vi "Game_Board_Click.vi"(0 "Context":T1={"Screen"=enum."Settings", "Settings"=[0, 0, 1, 1], "Board"={"Grid"=array15x15[225 elements], "Move History"=[], "Last Move"={"Row"=-1, "Col"=-1, "Stone"=enum."Empty"}}, "Status"=enum."Idle", "Game ID"=0, "Player Stone"=enum."Black", "Hover"={"Row"=-1, "Col"=-1, "Stone"=enum."Empty"}, "Hover Button"=-1, "Win Line"=[], "Score 1"=0, "Score 2"=0, "Draws"=0, "Status Text"="", "Status Color"=0}, 5 "Row":i32=-1, 7 "Col":i32=-1, 11 "error in":errorcluster) -> (4 "Context out":T1={"Screen"=enum."Settings", "Settings"=[0, 0, 1, 1], "Board"={"Grid"=array15x15[225 elements], "Move History"=[], "Last Move"={"Row"=-1, "Col"=-1, "Stone"=enum."Empty"}}, "Status"=enum."Idle", "Game ID"=0, "Player Stone"=enum."Black", "Hover"={"Row"=-1, "Col"=-1, "Stone"=enum."Empty"}, "Hover Button"=-1, "Win Line"=[], "Score 1"=0, "Score 2"=0, "Draws"=0, "Status Text"="", "Status Color"=0}, 6 "Need AI":bool, 15 "error out":errorcluster)   [LabVIEW 2026]
doc: "바둑판 (Row,Col) 클릭 처리. 2인 플레이는 수순(짝/홀)으로 흑/백 결정, AI 대전은 Player Stone.\n승/무/금수/차례 문구와 점수를 갱신하고, AI 대전에서 게임이 계속되면 Need AI = True."
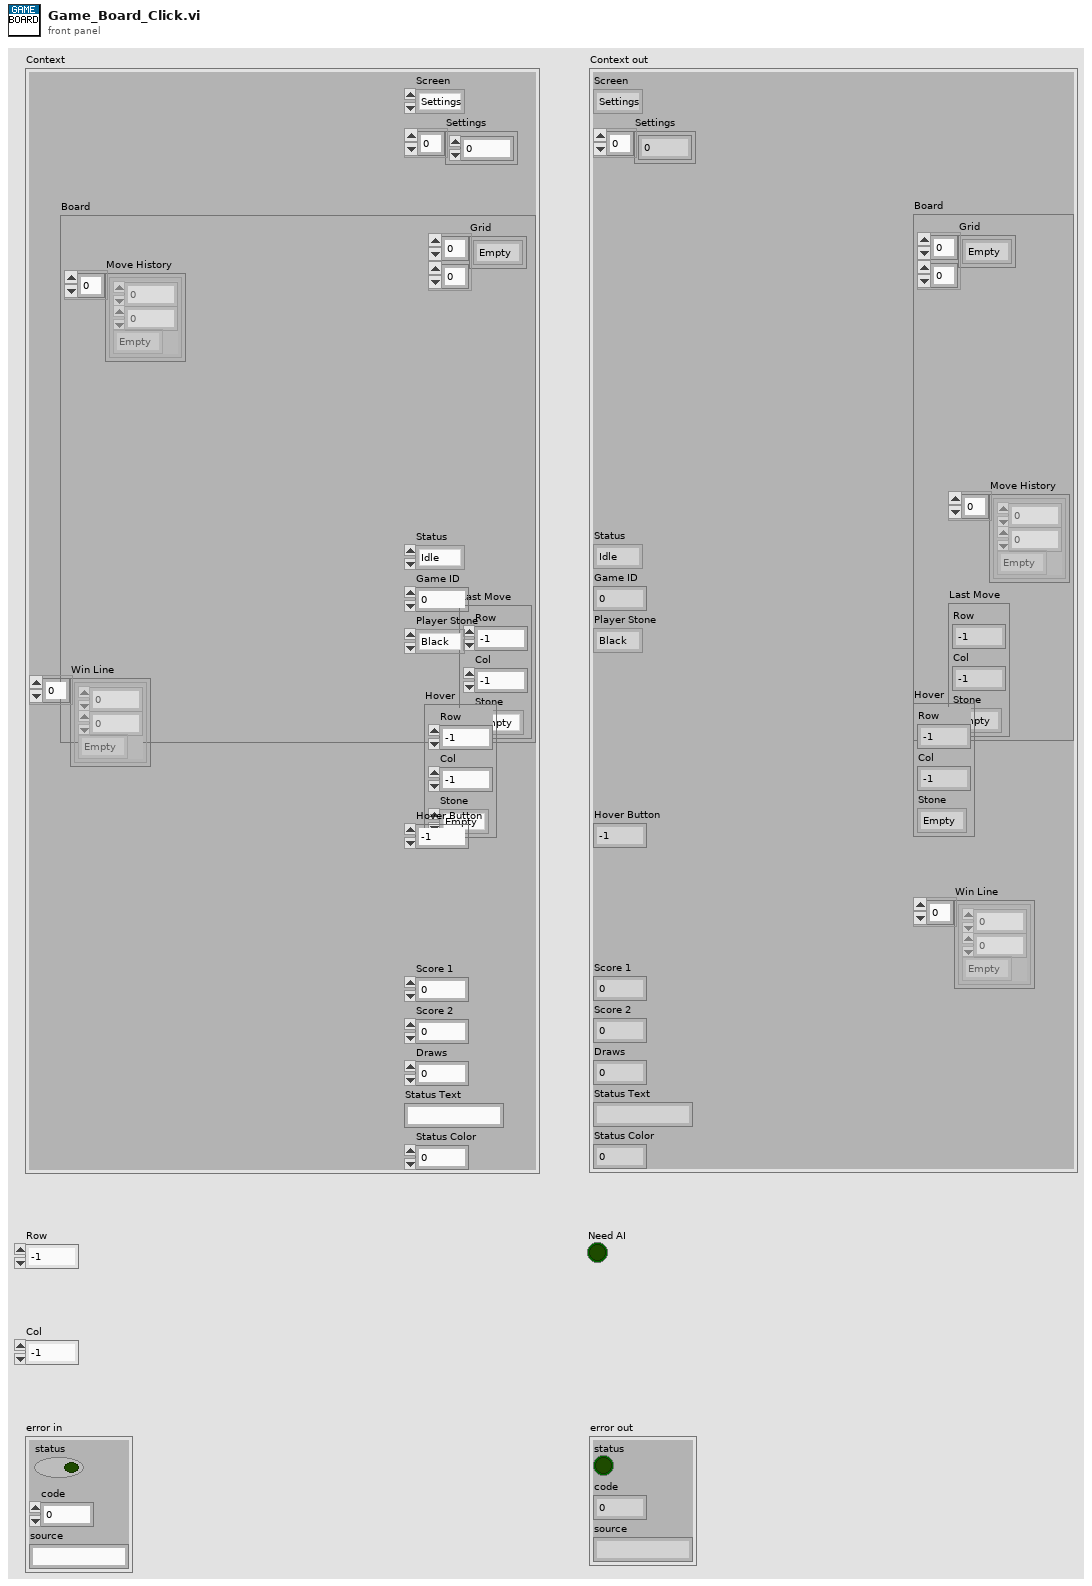
[diagram p1: front panel]
types:
  T1 = cluster{"Screen":enum16{"Settings", "Game"}, "Settings":i32[], "Board":cluster{"Grid":enum8{"Empty", "Black", "White"}[][], "Move History":cluster{"Row":i32, "Col":i32, "Stone":enum8{"Empty", "Black", "White"}}[], "Last Move":cluster{"Row":i32, "Col":i32, "Stone":enum8{"Empty", "Black", "White"}}}, "Status":enum16{"Idle", "Player Turn", "AI Thinking", "Game Over"}, "Game ID":u32, "Player Stone":enum8{"Empty", "Black", "White"}, "Hover":cluster{"Row":i32, "Col":i32, "Stone":enum8{"Empty", "Black", "White"}}, "Hover Button":i32, "Win Line":cluster{"Row":i32, "Col":i32, "Stone":enum8{"Empty", "Black", "White"}}[], "Score 1":i32, "Score 2":i32, "Draws":i32, "Status Text":string, "Status Color":u32}
  T2 = enum16{"Idle", "Player Turn", "AI Thinking", "Game Over"}
  T3 = cluster{"Row":i32, "Col":i32, "Stone":enum8{"Empty", "Black", "White"}}
  T4 = enum8{"None", "Double Three", "Double Four", "Overline"}
  T5 = cluster{"Grid":enum8{"Empty", "Black", "White"}[][], "Move History":cluster{"Row":i32, "Col":i32, "Stone":enum8{"Empty", "Black", "White"}}[], "Last Move":cluster{"Row":i32, "Col":i32, "Stone":enum8{"Empty", "Black", "White"}}}
  T6 = cluster{"Row":i32, "Col":i32, "Stone":enum8{"Empty", "Black", "White"}}[]
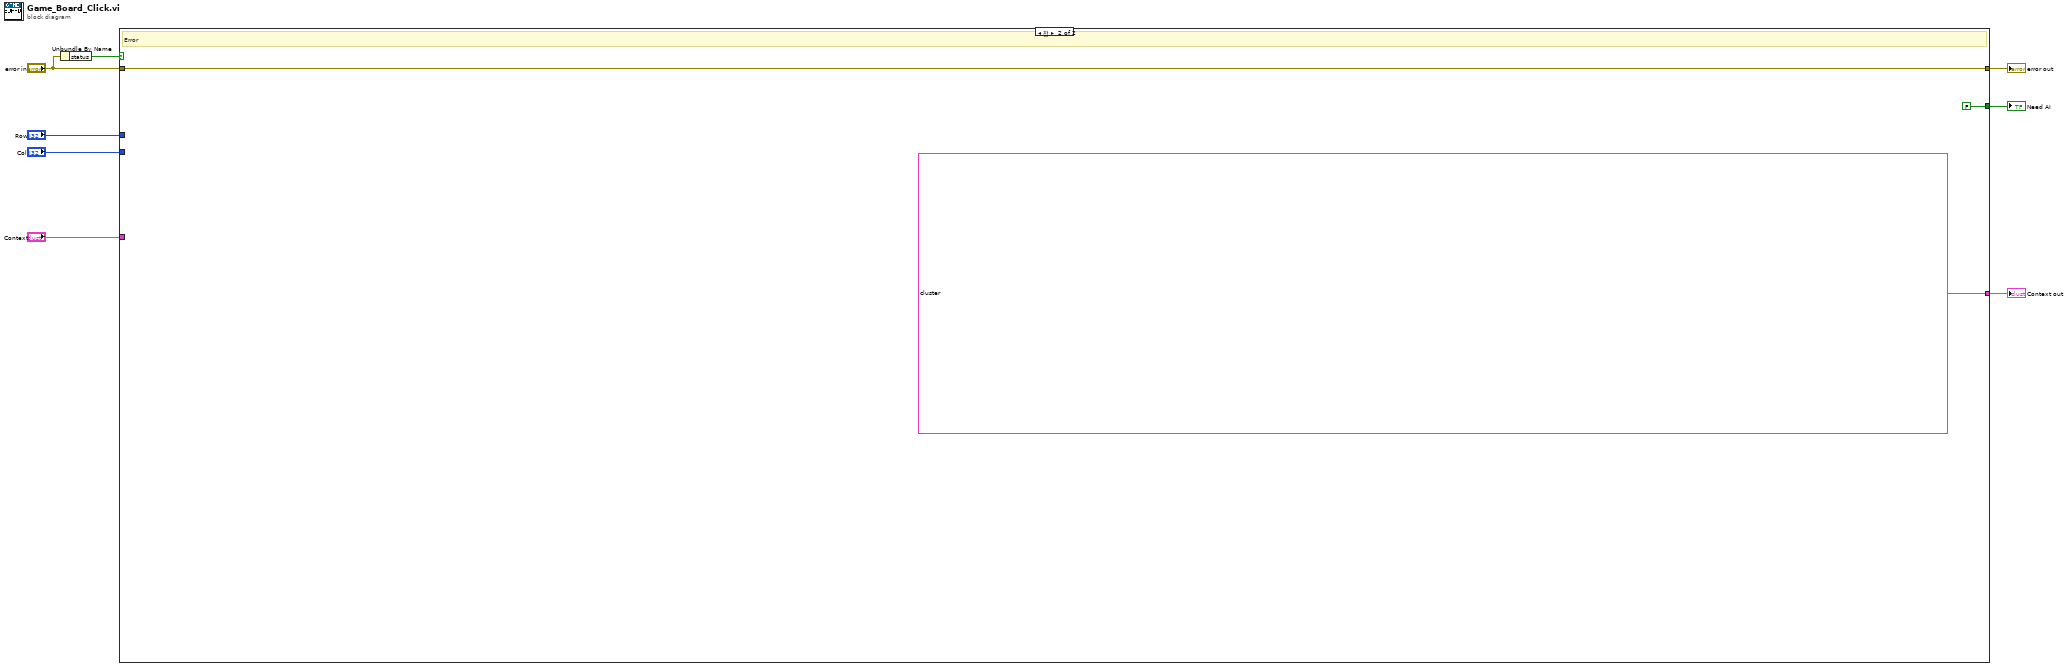
[diagram p0: block diagram]
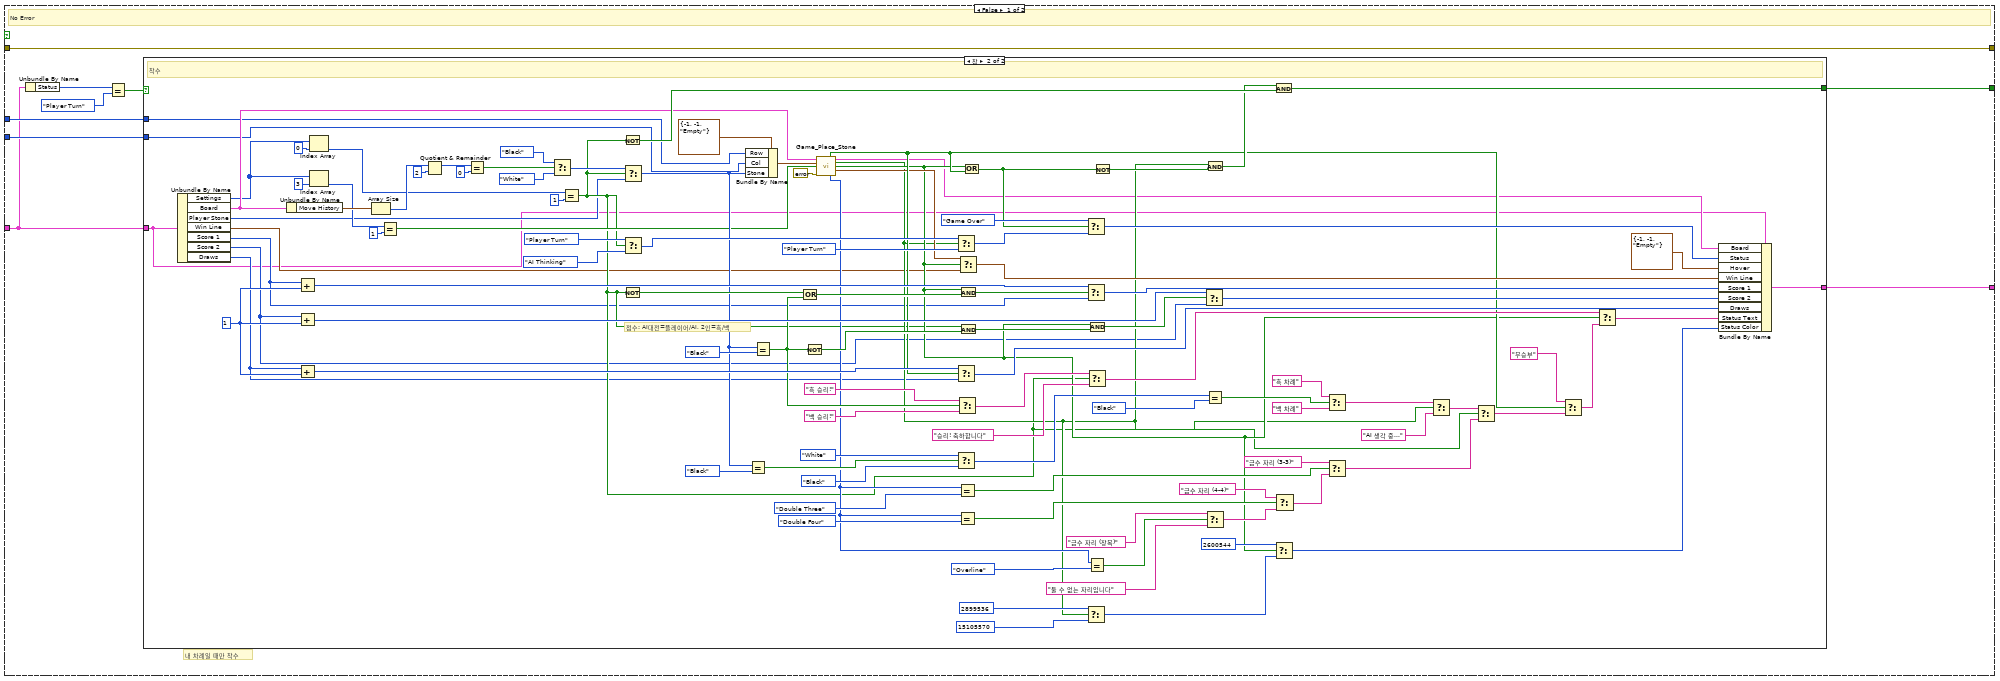
[diagram p2: hidden frame]
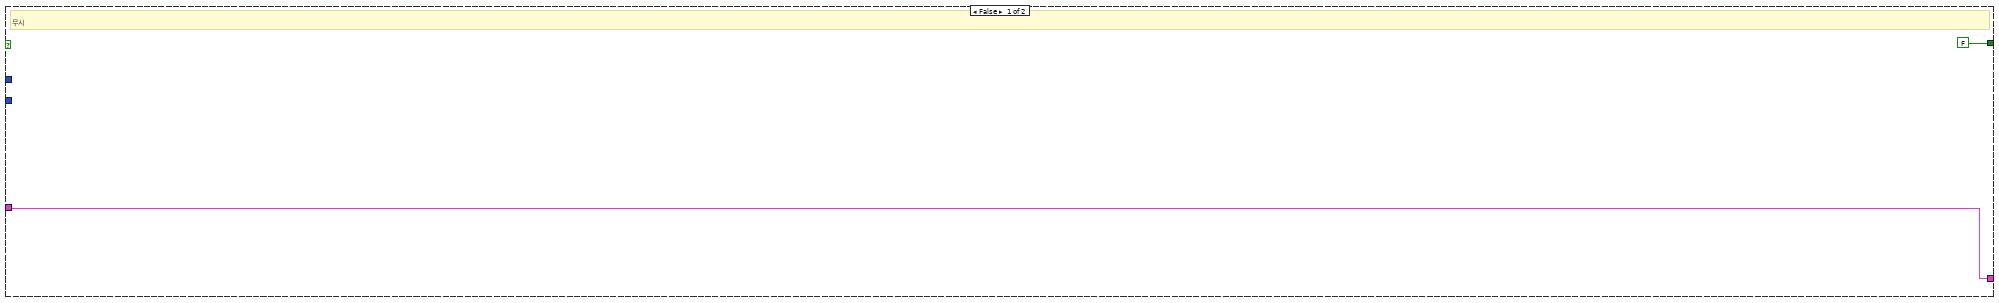
[diagram p3: hidden frame]
diagram:
  n1 = Unbundle By Name("error in") -> ("status"=w5:bool)
  n2 = case shown="참" w5 {
    tunnel: "Context" -> [w9 _]
    tunnel: "Row" -> [w10 _]
    tunnel: "Col" -> [w11 _]
    tunnel: "error in" -> [w12 w126]
    tunnel: [w12 w126] -> w8
    tunnel: [w17 FALSE] -> w7
    tunnel: [w16 T1 {"Screen"=enum."Settings", "Settings"=[0, 0, 1, 1], "Board"={"Grid"=array15x15[225 elements], "Move History"=[], "Last Move"={"Row"=-1, "Col"=-1, "Stone"=enum."Empty"}}, "Status"=enum."Idle", "Game ID"=0, "Player Stone"=enum."Black", "Hover"={"Row"=-1, "Col"=-1, "Stone"=enum."Empty"}, "Hover Button"=-1, "Win Line"=[], "Score 1"=0, "Score 2"=0, "Draws"=0, "Status Text"="", "Status Color"=0}] -> w6
    frame False {
      # "내 차례일 때만 착수"
      # "No Error"
      n3 = Unbundle By Name(w9) -> ("Status"=w13:T2)
      n4 = Equal?(x=w13, y=T2."Player Turn") -> (x = y?=w15:bool)
      n5 = case shown="참" w15 {
        tunnel: w9 -> [w18 w20]
        tunnel: w10 -> [_ w21]
        tunnel: w11 -> [_ w22]
        tunnel: [FALSE w61] -> w17
        tunnel: [w18 w125] -> w16
        frame False {
          # "무시"
        }
        frame True {
          w64 = 1
          # "점수: AI대전=플레이어/AI, 2인=흑/백"
          # "착수"
          n6 = Unbundle By Name(w20) -> ("Settings"=w23:i32[], "Board"=w24:T5, "Player Stone"=w25:enum8{"Empty", "Black", "White"}, "Win Line"=w26:T6, "Score 1"=w27:i32, "Score 2"=w28:i32, "Draws"=w29:i32)
          n7 = Unbundle By Name(w24) -> ("Move History"=w38:T6)
          n8 = Add(x=w27, y=w64) -> (x+y=w119:i32)
          n9 = Add(x=w28, y=w64) -> (x+y=w121:i32)
          n10 = Add(x=w29, y=w64) -> (x+y=w123:i32)
          n11 = Index Array(array=w23, index=0) -> (element=w31:i32)
          n12 = Index Array(array=w23, index=3) -> (element=w35:i32)
          n13 = Array Size(array=w38) -> (size(s)=w39:i32)
          n14 = Equal?(x=w35, y=1) -> (x = y?=w37:bool)
          n15 = Quotient & Remainder(x=w39, y=2) -> (x-y*floor(x/y)=w41:i32)  [unwired: 1 out]
          n16 = Equal?(x=w41, y=0) -> (x = y?=w43:bool)
          n17 = Select(t=enum8{"Empty", "Black", "White"}."Black", s=w43, f=enum8{"Empty", "Black", "White"}."White") -> (s? t:f=w46:enum8{"Empty", "Black", "White"})
          n18 = Equal?(x=w31, y=1) -> (x = y?=w33:bool)
          n19 = Not(x=w33) -> (.not. x?=w60:bool)
          n20 = Not(x=w33) -> (.not. x?=w65:bool)
          n21 = Select(t=w46, s=w33, f=w25) -> (s? t:f=w47:enum8{"Empty", "Black", "White"})
          n22 = Select(t=T2."Player Turn", s=w33, f=T2."AI Thinking") -> (s? t:f=w74:T2)
          n23 = Bundle By Name(cluster=T3 {"Row"=-1, "Col"=-1, "Stone"=enum."Empty"}, "Row"=w21, "Col"=w22, "Stone"=w47) -> (w49:T3)
          n24 = Equal?(x=w47, y=enum8{"Empty", "Black", "White"}."Black") -> (x = y?=w97:bool)
          n25 = Equal?(x=w47, y=enum8{"Empty", "Black", "White"}."Black") -> (x = y?=w63:bool)
          n26 = Or(x=w65, y=w63) -> (x .or. y?=w66:bool)
          n27 = Not(x=w63) -> (.not. x?=w68:bool)
          n28 = call "Game_Place_Stone.vi"("Board State"=w24, "Move"=w49, "Renju"=w37, "error in"=errorcluster {"status"=FALSE, "code"=0, "source"=""}) -> ("Draw?"=w56:bool, "Board State out"=w51:T5, "Placed?"=w52:bool, "Win?"=w53:bool, "Win Line"=w54:T6, "Forbidden Reason"=w55:T4)  [unwired: 5 in, 1 out]
          n29 = Select(t=w74, s=w52, f=T2."Player Turn") -> (s? t:f=w76:T2)
          n30 = Select(t=w123, s=w56, f=w29) -> (s? t:f=w124:i32)
          n31 = Select(t=enum8{"Empty", "Black", "White"}."White", s=w97, f=enum8{"Empty", "Black", "White"}."Black") -> (s? t:f=w100:enum8{"Empty", "Black", "White"})
          n32 = Select(t="흑 승리!", s=w63, f="백 승리!") -> (s? t:f=w93:string)
          n33 = Equal?(x=w55, y=T4."Double Three") -> (x = y?=w79:bool)
          n34 = Equal?(x=w55, y=T4."Double Four") -> (x = y?=w82:bool)
          n35 = Select(t=w54, s=w53, f=w26) -> (s? t:f=w118:T6)
          n36 = And(x=w53, y=w66) -> (x .and. y?=w67:bool)
          n37 = And(x=w33, y=w68) -> (x .and. y?=w69:bool)
          n38 = Or(x=w53, y=w56) -> (x .or. y?=w57:bool)
          n39 = Select(t=T2."Game Over", s=w57, f=w76) -> (s? t:f=w77:T2)
          n40 = Select(t=w119, s=w67, f=w27) -> (s? t:f=w120:i32)
          n41 = Select(t=u32 2899536, s=w52, f=u32 15105570) -> (s? t:f=w115:u32)
          n42 = Select(t=w93, s=w33, f="승리! 축하합니다") -> (s? t:f=w95:string)
          n43 = Equal?(x=w55, y=T4."Overline") -> (x = y?=w85:bool)
          n44 = And(x=w53, y=w69) -> (x .and. y?=w70:bool)
          n45 = Not(x=w57) -> (.not. x?=w58:bool)
          n46 = Select(t=w121, s=w70, f=w28) -> (s? t:f=w122:i32)
          n47 = Equal?(x=w100, y=enum8{"Empty", "Black", "White"}."Black") -> (x = y?=w102:bool)
          n48 = Select(t="금수 자리 (장목)", s=w85, f="둘 수 없는 자리입니다") -> (s? t:f=w88:string)
          n49 = And(x=w52, y=w58) -> (x .and. y?=w59:bool)
          n50 = And(x=w59, y=w60) -> (x .and. y?=w61:bool)
          n51 = Select(t=u32 2600544, s=w53, f=w115) -> (s? t:f=w116:u32)
          n52 = Select(t="금수 자리 (4-4)", s=w82, f=w88) -> (s? t:f=w89:string)
          n53 = Select(t="흑 차례", s=w102, f="백 차례") -> (s? t:f=w105:string)
          n54 = Select(t="금수 자리 (3-3)", s=w79, f=w89) -> (s? t:f=w90:string)
          n55 = Select(t=w105, s=w33, f="AI 생각 중...") -> (s? t:f=w107:string)
          n56 = Select(t=w107, s=w52, f=w90) -> (s? t:f=w109:string)
          n57 = Select(t="무승부", s=w56, f=w109) -> (s? t:f=w110:string)
          n58 = Select(t=w95, s=w53, f=w110) -> (s? t:f=w111:string)
          n59 = Bundle By Name(cluster=w20, "Board"=w51, "Status"=w77, "Hover"=T3 {"Row"=-1, "Col"=-1, "Stone"=enum."Empty"}, "Win Line"=w118, "Score 1"=w120, "Score 2"=w122, "Draws"=w124, "Status Text"=w111, "Status Color"=w116) -> (w125:T1)
        }
      }
    }
    frame True {
      # "Error"
    }
  }
  "Context out" <- w6
  "Need AI" <- w7
  "error out" <- w8
